vi "set NR Modulation.vi"(8 "error in (no error)":errorcluster, 10 "Modulation":T1, 11 "Anritsu Call Box_Implement in":refnum<class "Anritsu Call Box_Implement.lvclass">) -> (0 "error out":errorcluster, 3 "Anritsu Call Box_Implement out":refnum<class "Anritsu Call Box_Implement.lvclass">)   [LabVIEW 2023, in "ANRITSU Call Box.lvlib" / "Anritsu Call Box_Implement.lvclass"]
uses:
  Anritsu Call Box_Implement.lvclass
  Type Definition/NR Modulation Type.ctl
  Anritsu Call Box_Implement.lvclass/Anritsu Call Box_Implement.ctl
  NR/NR.lvclass
  ANRITSU Call Box.lvlib
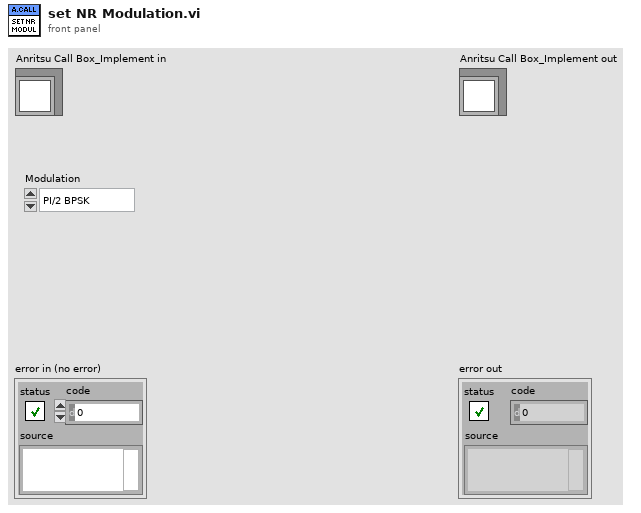
[diagram p1: front panel]
types:
  T1 = typedef "ANRITSU Call Box.lvlib/NR Modulation Type.ctl" = enum16{"PI/2 BPSK", "QPSK", "16QAM", "64QAM", "256QAM"}
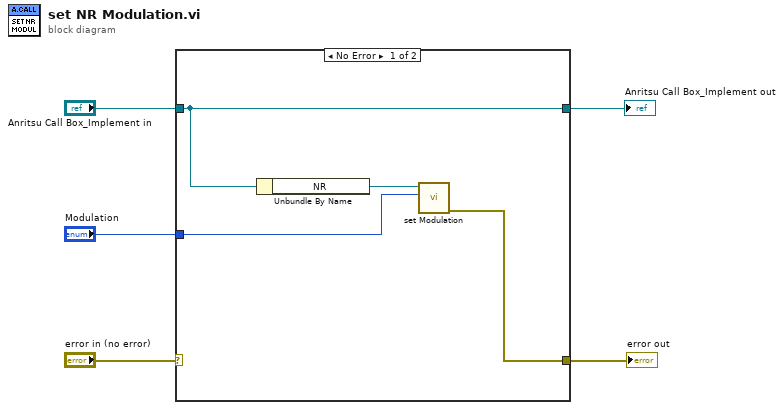
[diagram p0: block diagram]
diagram:
  n1 = case shown="No Error" "error in (no error)" {
    selector: "error in (no error)" -> [_ w10]
    tunnel: "Anritsu Call Box_Implement in" -> [w9 w11]
    tunnel: [w9 w11] -> w4
    tunnel: [w7 w10] -> w2
    tunnel: "Modulation" -> [w6 _]
    frame No Error {
      n2 = Unbundle By Name(w9) -> ("NR"=w8:refnum<class "NR.lvclass">)
      n3 = call "set Modulation.vi"("Modulation"=w6, "NR in"=w8) -> ("error out"=w7:errorcluster)  [unwired: 8 in, 1 out]
    }
    frame Error {
    }
  }
  "error out" <- w2
  "Anritsu Call Box_Implement out" <- w4
